vi "Handle Event.vi"(8 "error in (no error)":errorcluster, 9 "Controller in":refnum<class "Controller.lvclass">, 10 "Event Data":refnum<class "Event.lvclass">, 11 "Abstract Event Handler for Controller in":refnum<class "Abstract Event Handler for Controller.lvclass">) -> (0 "error out":errorcluster, 1 "Controller out":refnum<class "Controller.lvclass">, 3 "Abstract Event Handler for Controller out":refnum<class "Abstract Event Handler for Controller.lvclass">)   [LabVIEW 2023, in "MVC Actors.lvlib" / "Abstract Event Handler for Controller.lvclass"]
doc: "Abstract method to be implemented in the concrete subcalss to handle <b>Controller</b> events. Within this method the input <b>Event</b> should be cast to the expected concrete implementation and used as argument to the <b>Controller</b> method designated to handle the specific <b>Event</b>."
uses:
  Abstract Event Handler for Controller.lvclass
  Event/Event.lvclass
  Controller/Controller.lvclass
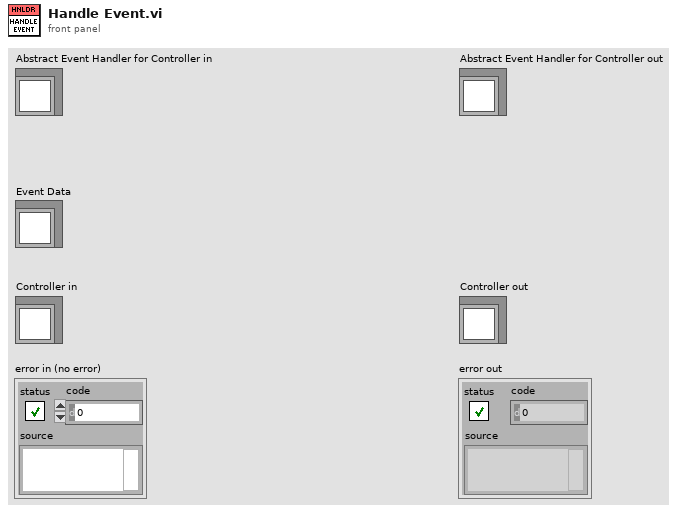
[diagram p1: front panel]
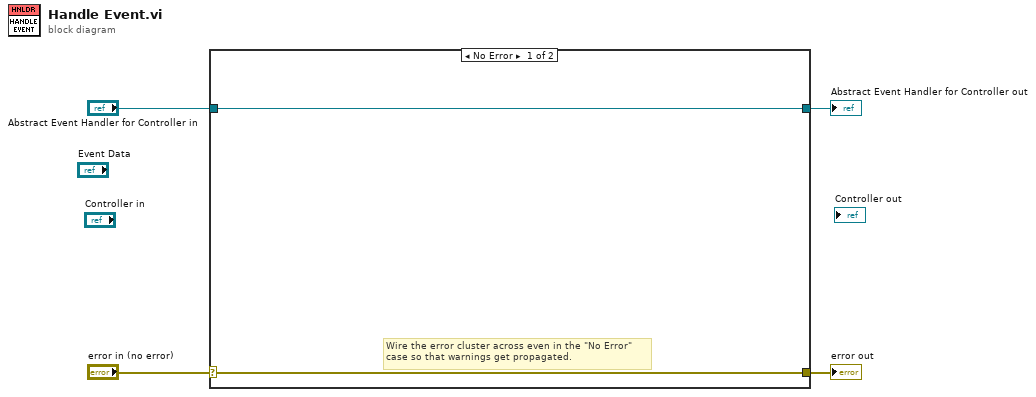
[diagram p0: block diagram]
diagram:
  n1 = case shown="No Error" "error in (no error)" {
    selector: "error in (no error)" -> [w5 w8]
    tunnel: [w5 w8] -> w3
    tunnel: [w6 w7] -> w1
    tunnel: "Abstract Event Handler for Controller in" -> [w6 w7]
    frame No Error {
      # "Wire the error cluster across even in the \"No Error\"\ncase so that warnings get propagated."
    }
    frame Error {
    }
  }
  "error out" <- w3
  "Abstract Event Handler for Controller out" <- w1
